vi "Day 22.vi"() -> ()   [LabVIEW 2021]
uses:
  <vilib>/Utility/file.llb/Read Delimited Spreadsheet (string).vi
  <vilib>/regexp/Match Regular Expression.xnode
panel:
  out "Cubes On":u64
  out "Array":cluster{bool, i32[]}[](array[cluster])
  in  "Input File":enum32{"example input", "input"}(radio)
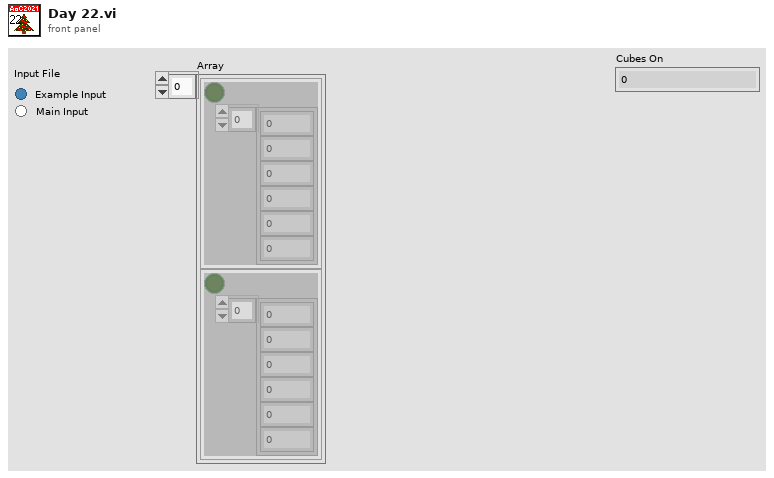
[diagram p1: front panel]
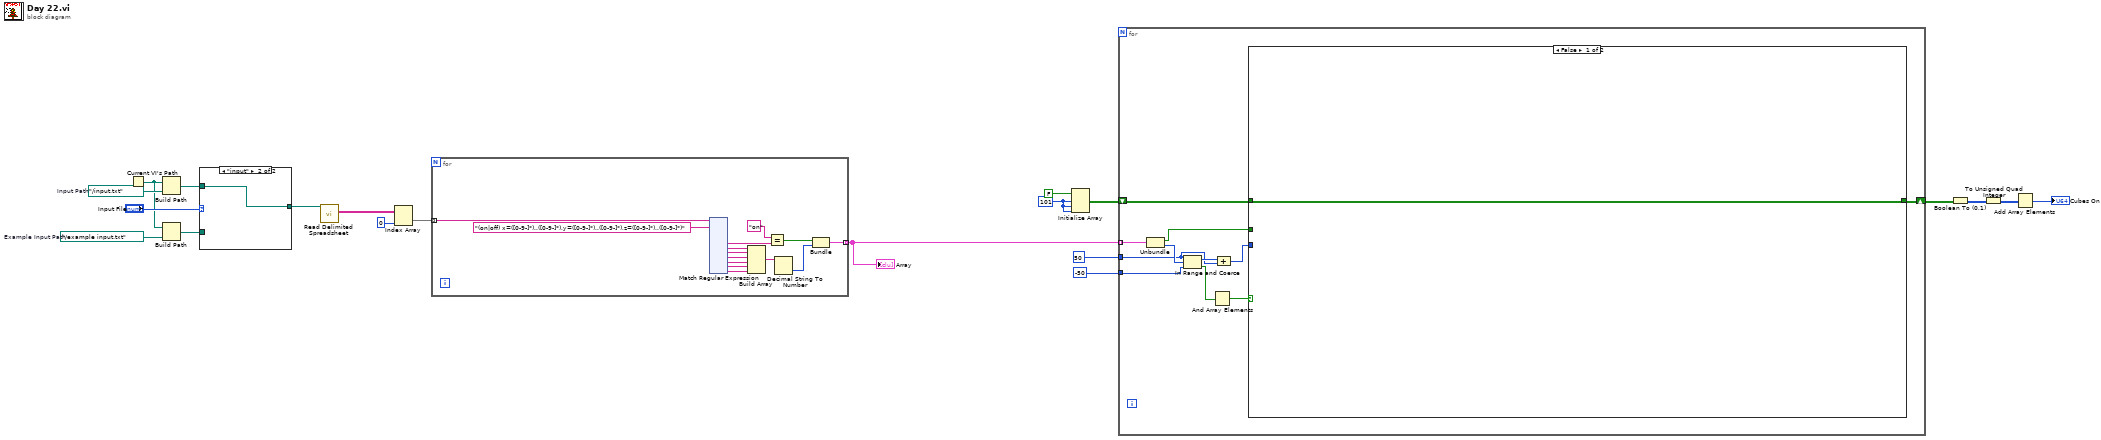
[diagram p0: block diagram]
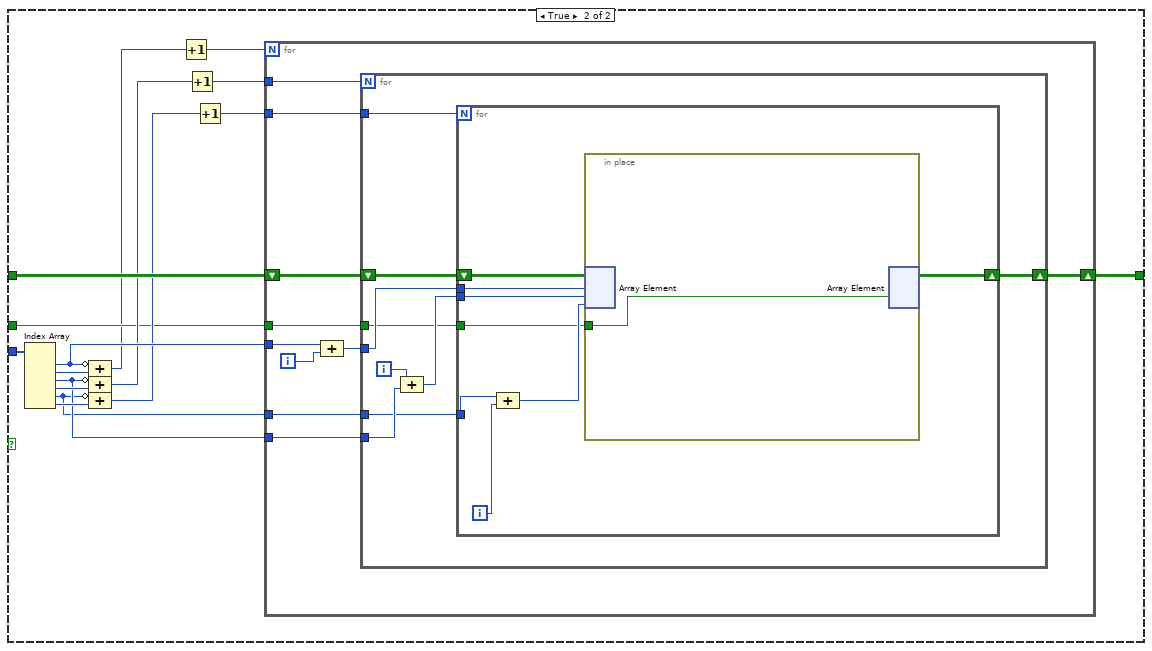
[diagram p2: hidden frame]
diagram:
  w9 = 101
  w19 = path "../example input.txt"  # Example Input Path
  w20 = path "../input.txt"  # Input Path
  n1 = Current VI's Path() -> (path=w14:path)
  n2 = Build Path(base path=w14, name or relative path=w20) -> (appended path=w17:path)
  n3 = Build Path(base path=w14, name or relative path=w19) -> (appended path=w16:path)
  n4 = case shown="\"input\"" "Input File" {
    tunnel: w17 -> [_ w22]
    tunnel: w16 -> [w21 _]
    tunnel: [w21 w22] -> w15
    frame "example input" {
    }
    frame "input" {
    }
  }
  n5 = call-poly <vilib>:"Read Delimited Spreadsheet.vi"("file path (dialog if empty)"=w15) -> ("all rows"=w13:string[][])  [unwired: 9 in, 5 out]
  n6 = Index Array(array=w13, index (col)=0 ("disabled index (col)")) -> (element=w11:string[])  [unwired: 1 in]
  n7 = for {
    tunnel: w11 -> [w36] mode=indexing
    tunnel: [w23] -> w4 mode=indexing
    n8 = xnode "Match Regular Expression"("input string"=w36, "regular expression"="(on|off) x=([0-9-]*)..([0-9-]*),y=([0-9-]*)..([0-9-]*),z=([0-9-]*)..([0-9-]*)") -> ("submatch 1"=w34:string, "submatch 2"=w31:string, "submatch 3"=w30:string, "submatch 4"=w29:string, "submatch 5"=w28:string, "submatch 6"=w27:string, "submatch 7"=w26:string)  [unwired: 4 in, 5 out]
    n9 = Build Array(w31, w30, w29, w28, w27, w26) -> (w25:string[])
    n10 = Equal?(x="on", y=w34) -> (x = y?=w32:bool)
    n11 = Decimal String To Number(string=w25) -> (number=w24:i32[])  [unwired: 2 in, 1 out]
    n12 = Bundle(w32, w24) -> (w23:cluster{bool, i32[]})  [unwired: 1 in]
  }
  "Array" <- w4
  n13 = Initialize Array(FALSE, w9, w9, w9) -> (w8:bool[][][])
  n14 = for {
    tunnel: w4 -> [w172] mode=indexing
    shift-right: [w170] -> w7
    shift-left: w8 -> [w171]
    tunnel: 50 -> [w164]
    tunnel: -50 -> [w165]
    n15 = Unbundle(w172) -> (w169:bool, w168:i32[])
    n16 = In Range and Coerce(upper limit=w164, x=w168, lower limit=w165) -> (coerced(x)=w167:i32[], In Range?=w163:bool[])
    n17 = And Array Elements(Boolean array=w163) -> (logical AND=w162:bool)
    n18 = Compound Arithmetic op=ADD(w167, w164) -> (w166:i32[])
    n19 = case shown="False" w162 {
      tunnel: w171 -> [w173 w186]
      tunnel: [w173 w185] -> w170
      tunnel: w169 -> [_ w179]
      tunnel: w166 -> [_ w178]
      frame False {
      }
      frame True {
        n20 = Index Array(array=w178) -> (element #1=w184:i32, element #2=w189:i32, element #3=w182:i32, element #4=w188:i32, element #5=w180:i32, element #6=w187:i32)  [unwired: 6 in]
        n21 = Compound Arithmetic op=ADD(invert w184, w189) -> (w177:i32)
        n22 = Compound Arithmetic op=ADD(invert w182, w188) -> (w183:i32)
        n23 = Compound Arithmetic op=ADD(invert w180, w187) -> (w181:i32)
        n24 = Increment(x=w177) -> (x+1=w176:i32)
        n25 = Increment(x=w183) -> (x+1=w175:i32)
        n26 = Increment(x=w181) -> (x+1=w174:i32)
        n27 = for {
          N: w176 -> [_]
          shift-right: [w193] -> w185
          shift-left: w186 -> [w199]
          tunnel: w184 -> [w198]
          tunnel: w175 -> [w196]
          tunnel: w182 -> [w195]
          tunnel: w174 -> [w192]
          tunnel: w180 -> [w191]
          tunnel: w179 -> [w190]
          i -> [w197]
          n28 = Compound Arithmetic op=ADD(w198, w197) -> (w194:i32)
          n29 = for {
            N: w196 -> [_]
            shift-right: [w203] -> w193
            shift-left: w199 -> [w208]
            tunnel: w195 -> [w205]
            tunnel: w194 -> [w207]
            tunnel: w192 -> [w202]
            tunnel: w191 -> [w201]
            tunnel: w190 -> [w200]
            i -> [w206]
            n30 = Compound Arithmetic op=ADD(w206, w205) -> (w204:i32)
            n31 = for {
              N: w202 -> [_]
              tunnel: w207 -> [w215]
              tunnel: w204 -> [w214]
              shift-right: [w213] -> w203
              shift-left: w208 -> [w216]
              tunnel: w201 -> [w211]
              tunnel: w200 -> [w209]
              i -> [w212]
              n32 = Compound Arithmetic op=ADD(w211, w212) -> (w210:i32)
              n33 = in-place {
                in-place-border: w209 -> [w217]
                n34 = in-place-array #1(w216, w215, w214, w210) -> ()  [unwired: 1 out]
                n35 = in-place-array #1(w217) -> (w213:bool[][][])  [unwired: 3 out]
              }
            }
          }
        }
      }
    }
  }
  n36 = Boolean To (0,1)(Boolean=w7) -> (0, 1=w6:i16[][][])
  n37 = To Unsigned Quad Integer(1:w6) -> (0:w1:u64[][][])
  n38 = Add Array Elements(numeric array=w1) -> (sum=→"Cubes On":u64)
